vi "Receive Message.vi"(6 "priority":i32, 10 "Async Methods Actor in":refnum<class "Async Methods Actor.lvclass">, 11 "Message in":refnum<class "Message.lvclass">) -> (0 "error out":errorcluster, 2 "Async Actor out":refnum<class "Actor.lvclass">)   [LabVIEW 2026, in "Async Methods Actor.lvlib" / "Async Methods Actor.lvclass"]
doc: "This VI should be overriden ONLY if you are creating a proxy actor for remote transmission. If you are, override this VI to transmit the received message to a new destination, maintaining the given priority."
uses:
  Async Methods Actor.lvclass
  <vilib>/ActorFramework/Message/Message.lvclass
  <vilib>/ActorFramework/Actor/Actor.lvclass
  C:/Program Files/National Instruments/LabVIEW 2026/vi.lib/ActorFramework/Actor/Actor.lvclass
  Async Methods Actor Messages/Async Message/Async Message.lvclass
  Async Methods Actor.lvclass/Async Methods Actor.ctl
  Async Methods Actor Messages/Async Message/Async Message.lvclass/Async Message.ctl
  Add Async Message to Map.vi
  Async Methods Actor Messages/Async Message/Read Async Call Method.vi
  Async Methods Actor Messages/Async Message/Read VI Refnum Lifetime.vi
  Write Async Message Execution Status Map.vi
  Async Methods Actor Messages/Async Message/Read FQN.vi
  Write Async Message Execution Status Map.vi/3adbf29e-89d7-4ecb-a2bd-8a8b89d527f8.vi
  Get VI FQN.vi
  <vilib>/Utility/LVClass/Get LV Class Path.vi
  <vilib>/ActorFramework/Actor Framework.lvlib
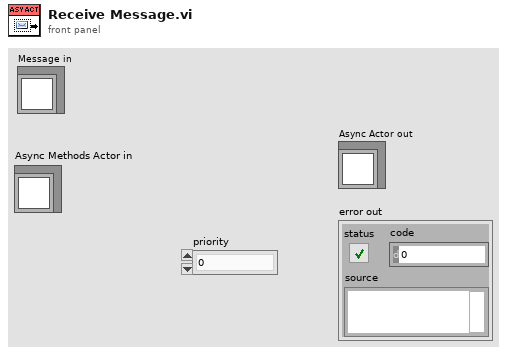
[diagram p1: front panel]
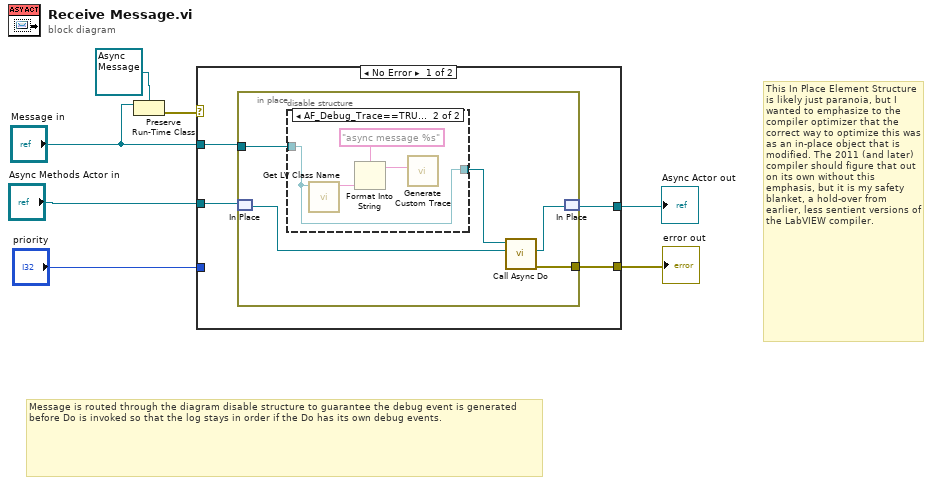
[diagram p0: block diagram]
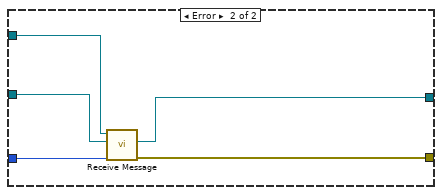
[diagram p3: hidden frame]
diagram:
  # "Message is routed through the diagram disable structure to guarantee the debug event is generated before Do is invoked so that the log stays in order if the Do has its own debug events."
  # "This In Place Element Structure is likely just paranoia, but I wanted to emphasize to the compiler optimizer that the correct way to optimize this was as an in-place object that is modified. The 2011 (and later) compiler should figure that out on its own without this emphasis, but it is my safety blanket, a hold-over from earlier, less sentient versions of the LabVIEW compiler."
  n1 = Preserve Run-Time Class(object in="Message in", 2:refnum<class "Async Message.lvclass"> refnum ("Async Actor.lvlib:Async Message Msg.lvclass")) -> (error out=w1:errorcluster)  [unwired: 1 in, 1 out]
  n2 = case shown="No Error" w1 {
    tunnel: [w11 w24] -> w7
    tunnel: [w10 w23] -> w6
    tunnel: "Async Methods Actor in" -> [w9 w25]
    tunnel: "Message in" -> [w8 w26]
    tunnel: "priority" -> [_ w22]
    frame No Error {
      n3 = in-place {
        in-place-border: [w16] -> w10
        in-place-border: w8 -> [w13]
        n4 = in-place-match #1(w9) -> (w15:refnum<class "Async Methods Actor.lvclass">)
        n5 = disable-structure shown="AF_Debug_Trace==TRUE" {
          disable-tunnel: w13 -> [w17 w18]
          disable-tunnel: [w17 w18] -> w12
          frame condition #0 (active) {
          }
          frame condition #1 {
            n6 = call <vilib>:"Get LV Class Name.vi"("object"=w18) -> ("class name"=w21:string)  [unwired: 9 in, 1 out]
            n7 = Format Into String(format string="async message %s", w21) -> (resulting string=w19:string)  [unwired: 2 in, 1 out]
            n8 = call <vilib>:"Generate Custom Trace.vi"("Custom Action"=w19) -> ()  [unwired: 11 in]
          }
        }
        n9 = call "Call Async Do.vi"("Async Methods Actor in"=w15, "Message in"=w12) -> ("error out"=w16:errorcluster, "Async Methods Actor out"=w14:refnum<class "Async Methods Actor.lvclass">)  [unwired: 8 in]
        n10 = in-place-match #1(w14) -> (w11:refnum<class "Async Methods Actor.lvclass">)
      }
    }
    frame Error {
      n11 = call-parent "Receive Message.vi"("priority"=w22, "Actor in"=w25, "Message in"=w26) -> ("error out"=w23:errorcluster, "Actor out"=w24:refnum<class "Actor.lvclass">)  [unwired: 7 in]
    }
  }
  "error out" <- w6
  "Async Actor out" <- w7
